vi "GetChannels.vi"(8 "error in (no error)":errorcluster, 11 "object in":refnum<class "ChannelsManager.lvclass">) -> (0 "error out":errorcluster, 2 "Channls":refnum<class "Channel.lvclass">[](array[class]), 3 "object out":refnum<class "ChannelsManager.lvclass">)   [LabVIEW 2021, in "Channel.lvlib" / "ChannelsManager.lvlib" / "ChannelsManager.lvclass"]
doc: "Read the Channels"
uses:
  ChannelsManager.lvclass
  Channel_class/Channel.lvclass
  ChannelsManager.lvclass/ChannelsManager.ctl
  <vilib>/Utility/config.llb/NI_LVConfig.lvlib
  Channel.lvlib
panel:
  out "Array 2":errorcluster[](array[cluster])
  out "Array":bool[](array[boolean])
  out "section names":string[](array[string])
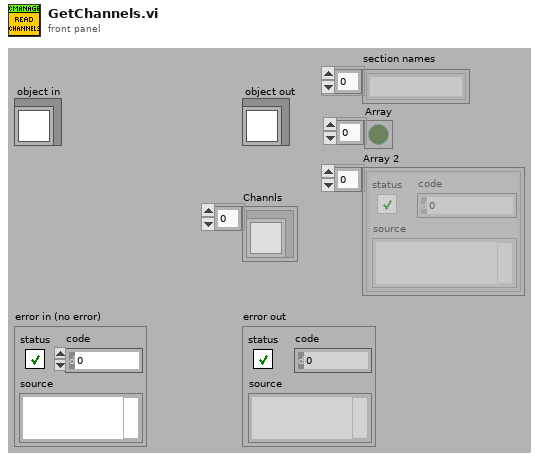
[diagram p1: front panel]
types:
  T1 = typedef "NI_LVConfig.lvlib/Config Data RefNum.ctl" = refnum<k1>
  T2 = cluster{"String":string, "Channel":refnum<class "Channel.lvclass">}
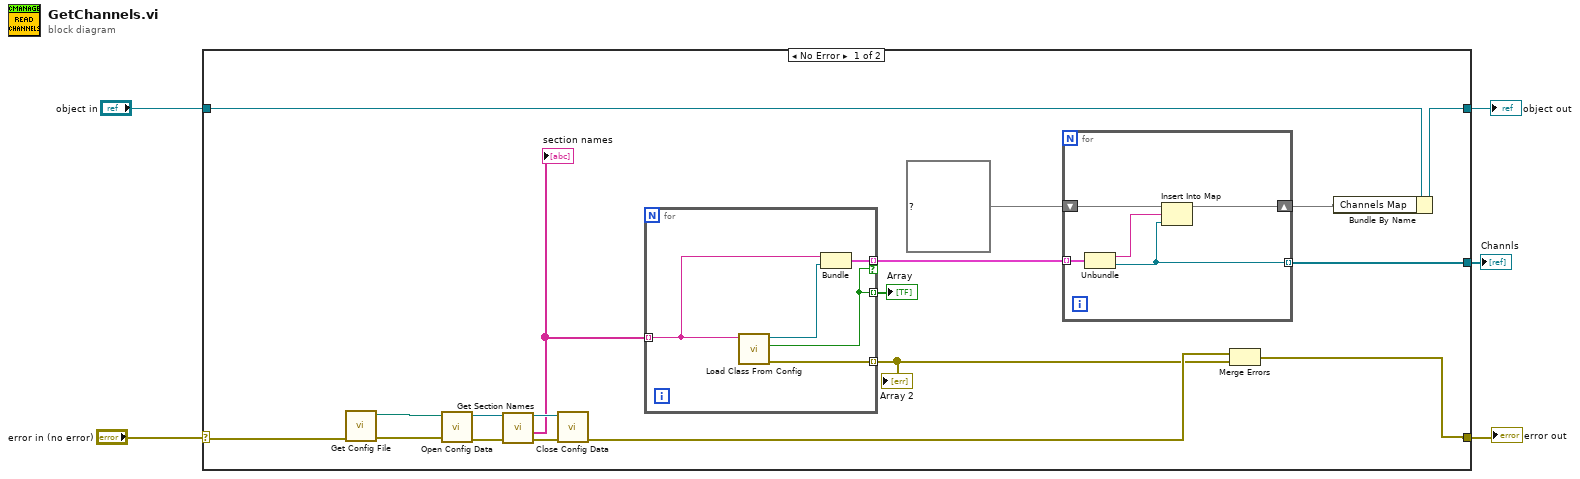
[diagram p0: block diagram]
diagram:
  n1 = case shown="No Error" "error in (no error)" {
    selector: "error in (no error)" -> [w12 w35]
    tunnel: [w15 w35] -> w4
    tunnel: [w10 w34] -> w2
    tunnel: "object in" -> [w23 w34]
    tunnel: [w7 _] -> w1
    frame No Error {
      n2 = call "Get Config File.vi"("error in (no error)"=w12) -> ("error out"=w13:errorcluster, "Config File"=w14:path)  [unwired: 9 in]
      n3 = call <vilib>:"Open Config Data.vi"("error in (no error)"=w13, "configuration file path"=w14) -> ("error out"=w19:errorcluster, "refnum"=w20:T1)  [unwired: 7 in, 1 out]
      n4 = call <vilib>:"Get Section Names.vi"("error in (no error)"=w19, "refnum"=w20) -> ("error out"=w22:errorcluster, "section names"=w18:string[], "refnum out"=w21:T1)  [unwired: 7 in]
      "section names" <- w18
      n5 = call <vilib>:"Close Config Data.vi"("error in (no error)"=w22, "refnum"=w21) -> ("error out"=w17:errorcluster)  [unwired: 8 in, 1 out]
      n6 = for {
        tunnel: w18 -> [w32] mode=indexing
        tunnel: [w33] -> w16 mode=indexing
        tunnel: [w30] -> w11 mode=indexing if=w29
        tunnel: [w29] -> w6 mode=indexing
        n7 = call "Load Class From Config.vi"("Name"=w32) -> ("error out"=w33:errorcluster, "Success"=w29:bool, "Channel"=w31:refnum<class "Channel.lvclass">)  [unwired: 8 in]
        n8 = Bundle("String"=w32, "Channel"=w31) -> (w30:T2)  [unwired: 1 in]
      }
      "Array" <- w6
      "Array 2" <- w16
      n9 = for {
        tunnel: w11 -> [w26] mode=indexing
        shift-right: [w27] -> w8
        shift-left: map{string, refnum<class "Channel.lvclass">} {} ("Channels Map") -> [w28]
        tunnel: [w24] -> w7 mode=indexing
        n10 = Unbundle(w26) -> ("String"=w25:string, "Channel"=w24:refnum<class "Channel.lvclass">)
        n11 = Insert Into Map(map in=w28, key=w25, value=w24) -> (map out=w27:map{string, refnum<class "Channel.lvclass">})  [unwired: 2 out]
      }
      n12 = Merge Errors(w17, w16) -> (w15:errorcluster)
      n13 = Bundle By Name(cluster=w23, "Channels Map"=w8) -> (w10:refnum<class "ChannelsManager.lvclass">)
    }
    frame Error {
    }
  }
  "error out" <- w4
  "object out" <- w2
  "Channls" <- w1
